vi "Host_NetworkStreams.vi"() -> ()   [LabVIEW 2025]
uses:
  <vilib>/dex/Flush And Wait Empty Condition.ctl
  <vilib>/Analysis/NI_AALBase.lvlib
panel:
  out "error out":errorcluster
  out "Sinus z RT":dbl[][](graph)
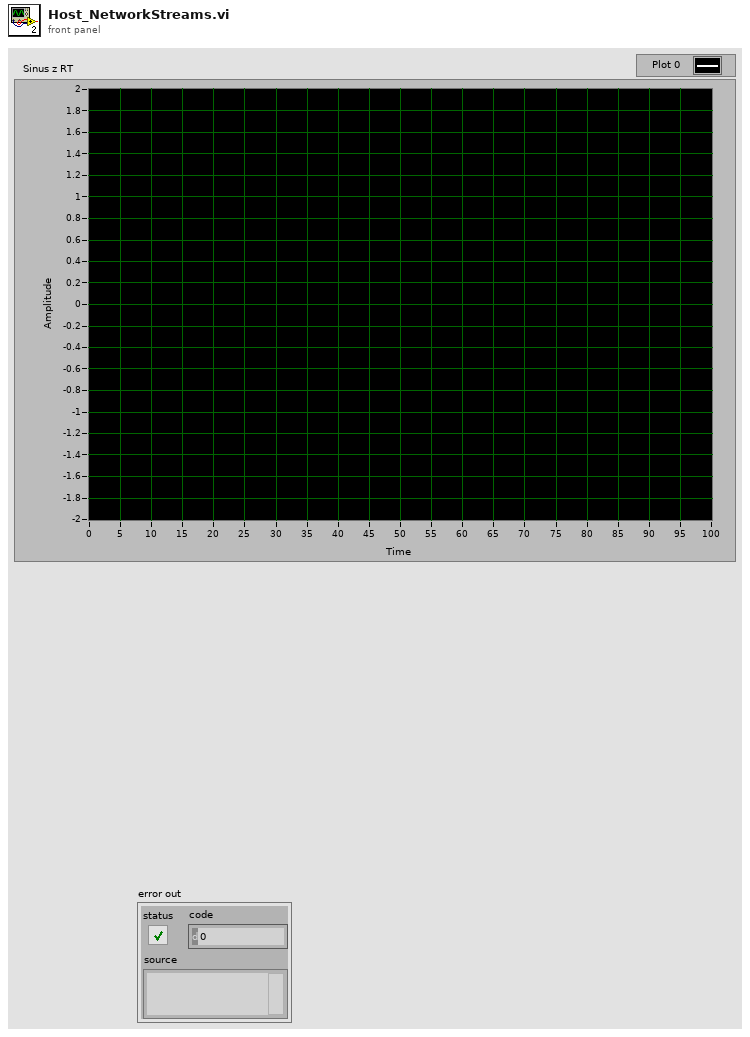
[diagram p1: front panel]
types:
  T1 = typedef "Flush And Wait Empty Condition.ctl" = u8
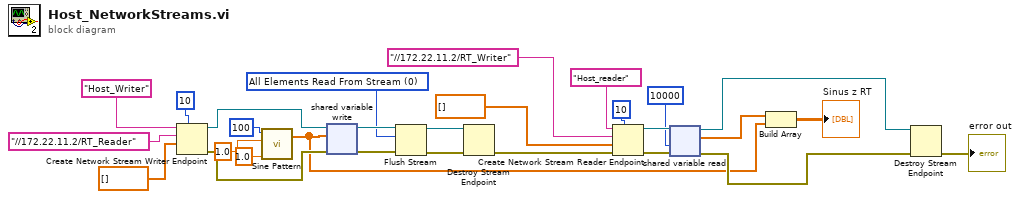
[diagram p0: block diagram]
diagram:
  w5 = T1 0 items=["All Elements Read From Stream", "All Elements Available for Reading"] ("wait condition")
  n1 = Create Network Stream Writer Endpoint(7:10 ("writer buffer size"), 9:dbl[] [], 10:"//172.22.11.2/RT_Reader" ("reader url"), 11:"Host_Writer" ("writer name")) -> (0:w20:errorcluster, 3:w21:refnum<k21>)  [unwired: 3 in]
  n2 = call <vilib>:"Sine Pattern.vi"("cycles"=1.0, "amplitude"=1.0, "samples"=100) -> ("Sinusoidal Pattern"=w2:dbl[])  [unwired: 1 in, 1 out]
  n3 = shared-variable-write(w21, w20, w2) -> (w19:refnum<k21>, w18:errorcluster)  [unwired: 1 in, 1 out]
  n4 = Flush Stream(8:w18, 10:w5, 11:w19) -> (0:w16:errorcluster, 3:w17:refnum<k21>)  [unwired: 1 in, 1 out]
  n5 = Destroy Stream Endpoint(8:w16, 11:w17) -> (0:w15:errorcluster)
  n6 = Create Network Stream Reader Endpoint(7:10 ("reader buffer size"), 8:w15, 9:dbl[] [], 10:"//172.22.11.2/RT_Writer" ("writer url"), 11:"Host_reader" ("reader name")) -> (0:w9:errorcluster, 3:w10:refnum<k21>)  [unwired: 2 in]
  n7 = shared-variable-read(w10, w9, 10000 ("timeout ms (-1)")) -> (w8:refnum<k21>, w7:errorcluster, w4:dbl[])  [unwired: 1 out]
  n8 = Build Array(w4, w2) -> (→"Sinus z RT":dbl[][])
  n9 = Destroy Stream Endpoint(8:w7, 11:w8) -> (0:→"error out":errorcluster)
